vi "串口读写 - DS.vi"(7 "寄存器地址":u8, 8 "错误输入（无错误）":errorcluster, 9 "写入数据":i32, 10 "写/读":T1, 11 "VISA输入":refnum<visa-resource-name>) -> (0 "错误输出":errorcluster, 1 "读取设备(n)":i32, 3 "VISA输出":refnum<visa-resource-name>)   [LabVIEW 2026, in "UI-距离测量.lvlib"]
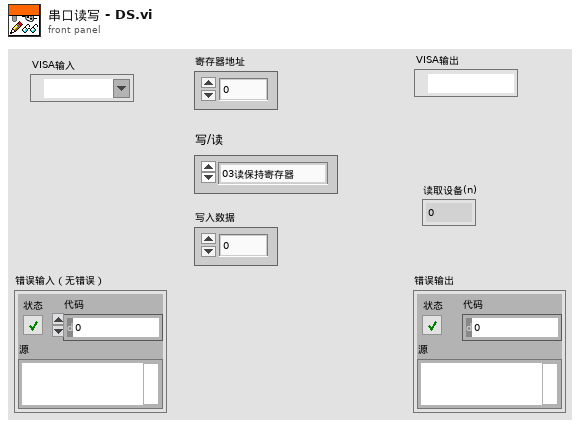
[diagram p1: front panel]
types:
  T1 = typedef "UI-距离测量.lvlib/读写指令类型.ctl" = enum16{"03读保持寄存器", "04读输入寄存器", "06写单个寄存器"}
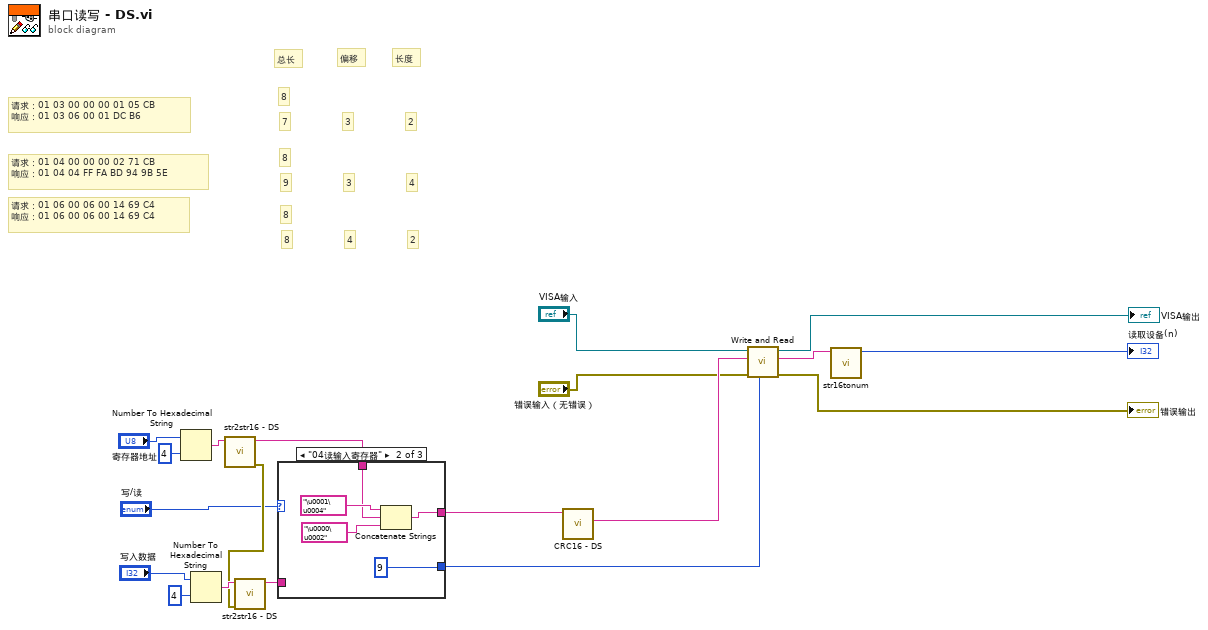
[diagram p0: block diagram]
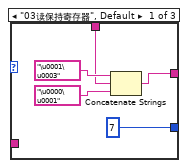
[diagram p2: hidden frame]
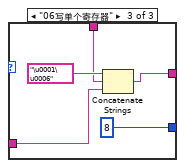
[diagram p3: hidden frame]
diagram:
  # "2"
  # "4"
  # "8"
  # "8"
  # "4"
  # "3"
  # "9"
  # "8"
  # "2"
  # "3"
  # "长度"
  # "偏移"
  # "7"
  # "总长"
  # "8"
  # "请求：01 06 00 06 00 14 69 C4\n响应：01 06 00 06 00 14 69 C4"
  # "请求：01 04 00 00 00 02 71 CB\n响应：01 04 04 FF FA BD 94 9B 5E"
  # "请求：01 03 00 00 00 01 05 CB\n响应：01 03 06 00 01 DC B6"
  n1 = Number To Hexadecimal String(1:i16 4 ("宽度(-)"), 2:"寄存器地址") -> (0:w15:string)
  n2 = Number To Hexadecimal String(1:i16 4 ("宽度(-)"), 2:"写入数据") -> (0:w18:string)
  n3 = call "str2str16 - DS.vi"("字符串"=w15) -> ("错误输出"=w13:errorcluster, "string"=w11:string)  [unwired: 9 in]
  n4 = call "str2str16 - DS.vi"("错误输入"=w13, "字符串"=w18) -> ("string"=w7:string)  [unwired: 8 in, 1 out]
  n5 = case shown="\"04读输入寄存器\"" "写/读" {
    tunnel: [w22 w27 w32] -> w10
    tunnel: w11 -> [w23 w28 w33]
    tunnel: [u32 7 ("读取字节数") u32 9 ("读取字节数") u32 8 ("读取字节数")] -> w8
    tunnel: w7 -> [_ _ w30]
    frame "03读保持寄存器", Default {
      n6 = Concatenate Strings("\u0001\u0003" ("Command"), w23, "\u0000\u0001" ("Command")) -> (w22:string)
    }
    frame "04读输入寄存器" {
      n7 = Concatenate Strings("\u0001\u0004" ("Command"), w28, "\u0000\u0002" ("Command")) -> (w27:string)
    }
    frame "06写单个寄存器" {
      n8 = Concatenate Strings("\u0001\u0006" ("Command"), w33, w30) -> (w32:string)
    }
  }
  n9 = call "CRC16 - DS.vi"("要校验的字符串（十六进制显示）"=w10) -> ("连接的字符串(16进制)"=w9:string)  [unwired: 9 in, 1 out]
  n10 = call "Write and Read.vi"("读取字节数"=w8, "错误输入（无错误）"="错误输入（无错误）", "Command"=w9, "VISA输入"="VISA输入") -> ("错误输出"=→"错误输出":errorcluster, "read buffer"=w2:string, "VISA输出"=→"VISA输出":refnum<visa-resource-name>)  [unwired: 5 in]
  n11 = call "str16tonum.vi"("字符串"=w2) -> ("数值"=→"读取设备(n)":i32)  [unwired: 10 in]
